vi "Choose Scale.vi"(9 "标尺引用":refnum<vi>, 10 "标尺选择":refnum<vi>, 11 "显示数据":T1[](array[typedef])) -> (2 "单位":string, 3 "名称":string)   [LabVIEW 2020, in "Data Viewer.lvlib" / "Data Viewer.lvclass"]
uses:
  Data Viewer.lvclass
  Data Serie--cluster.ctl
  Data Viewer.lvlib
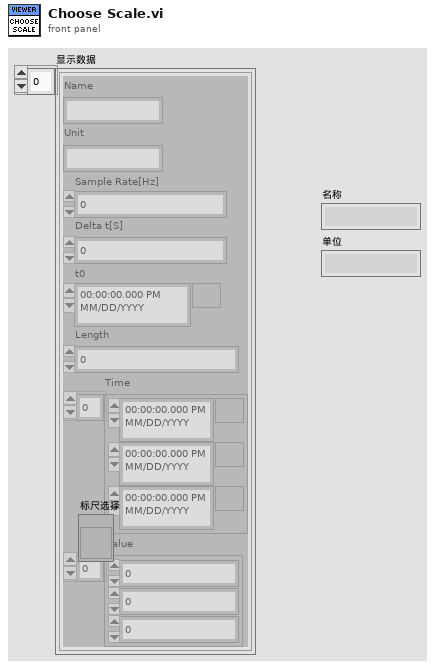
[diagram p1: front panel]
types:
  T1 = typedef "Data Viewer.lvlib/Data Serie--cluster.ctl" = cluster{"Name":string, "Unit":string, "Sample Rate[Hz]":dbl, "Delta t[S]":dbl, "t0":timestamp, "Length":i32, "Time":timestamp[], "Value":dbl[]}
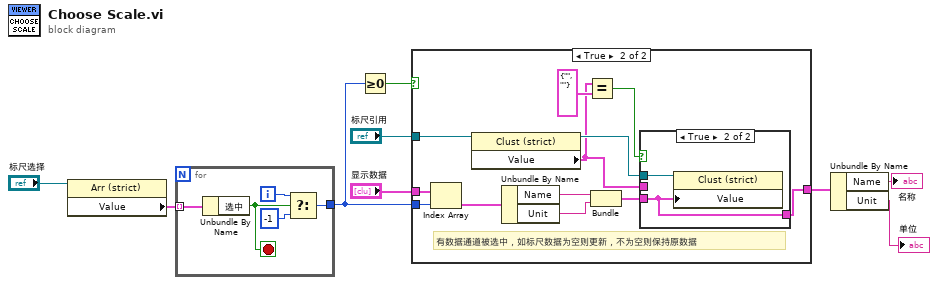
[diagram p0: block diagram]
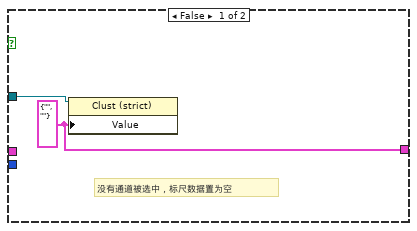
[diagram p2: hidden frame]
diagram:
  n1 = property class="Arr (strict)"(reference="标尺选择") -> ("Value"=w5:cluster{"选中":bool, "名称":string}[])  [unwired: 1 in, 2 out]
  n2 = for {
    tunnel: w5 -> [w14] mode=indexing
    tunnel: [w11] -> w7
    i -> [w12]
    stop <- w13 stop-if-true
    n3 = Unbundle By Name(w14) -> ("选中"=w13:bool)
    n4 = Select(t=w12, s=w13, f=-1) -> (s? t:f=w11:i32)
  }
  n5 = Greater Or Equal To 0?(x=w7) -> (x >= 0?=w6:bool)
  n6 = case shown="True" w6 {
    tunnel: w7 -> [_ w27]
    tunnel: "显示数据" -> [_ w28]
    tunnel: "标尺引用" -> [w16 w22]
    tunnel: [w15 w18] -> w3
    frame False {
      w15 = cluster{"名称":string, "单位":string} {"名称"="", "单位"=""} ("值")
      # "没有通道被选中，标尺数据置为空"
      n7 = property class="Clust (strict)"(reference=w16, "Value"=w15) -> ()  [unwired: 1 in, 2 out]
    }
    frame True {
      # "有数据通道被选中，如标尺数据为空则更新，不为空则保持原数据"
      n8 = Index Array(array=w28, index=w27) -> (element=w26:T1)
      n9 = property class="Clust (strict)"(reference=w22) -> (reference out=w19:refnum<vi>, "Value"=w17:cluster{"名称":string, "单位":string})  [unwired: 1 in, 1 out]
      n10 = Unbundle By Name(w26) -> ("Name"=w25:string, "Unit"=w24:string)
      n11 = Equal?(x=w17, y=cluster{"名称":string, "单位":string} {"名称"="", "单位"=""}) -> (x = y?=w20:bool)
      n12 = Bundle("Name"=w25, "Unit"=w24) -> (w23:cluster{"Name":string, "Unit":string})  [unwired: 1 in]
      n13 = case shown="True" w20 {
        tunnel: w23 -> [_ w30]
        tunnel: w19 -> [_ w31]
        tunnel: [w29 w30] -> w18
        tunnel: w17 -> [w29 _]
        frame False {
        }
        frame True {
          n14 = property class="Clust (strict)"(reference=w31, "Value"=w30) -> ()  [unwired: 1 in, 2 out]
        }
      }
    }
  }
  n15 = Unbundle By Name(w3) -> ("Name"=→"名称":string, "Unit"=→"单位":string)
